vi "VIH Dialog - Enter Web or Mail address.vi"(11 "Type":enum16{"Website", "Email"}(ring)) -> (0 "OK out":bool, 2 "Subject out":string, 3 "Address out":string)   [LabVIEW 2014]
doc: "::: VI Helpeks :::\nCopyright (c) 2000-2026 Konstantin Shifershteyn. All rights reserved."
uses:
  <vilib>/Utility/miscctls.llb/LVSelectionTypeDef.ctl
panel:
  in  "Subject":string
  in  "%Cancel":bool
  in  "%OK":bool
  in  "Address":string caption="Website URL"
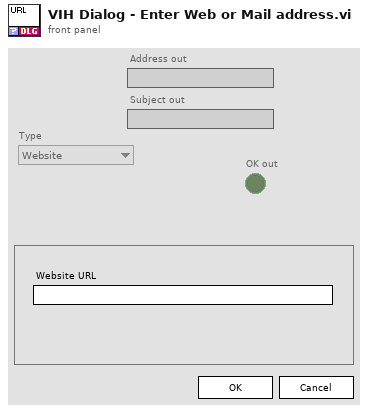
[diagram p1: front panel]
types:
  T1 = typedef "LVSelectionTypeDef.ctl" = cluster{"Selection Start":u32, "Selection End":u32}
  T2 = enum8{"Enabled", "Disabled", "Disabled and Grayed Out"}
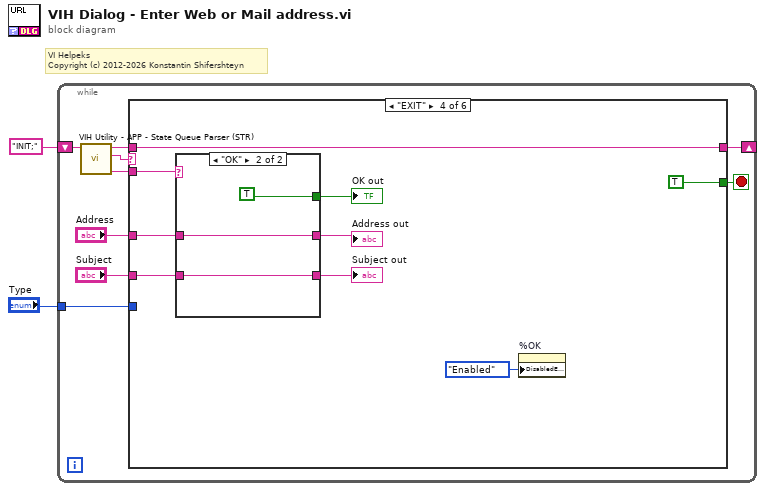
[diagram p0: block diagram]
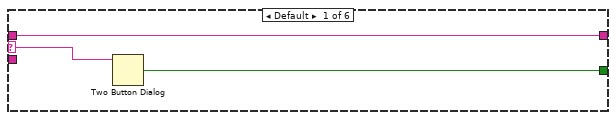
[diagram p2: hidden frame]
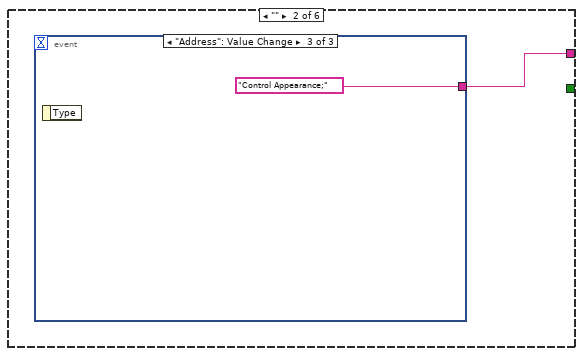
[diagram p3: hidden frame]
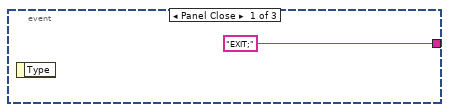
[diagram p4: hidden frame]
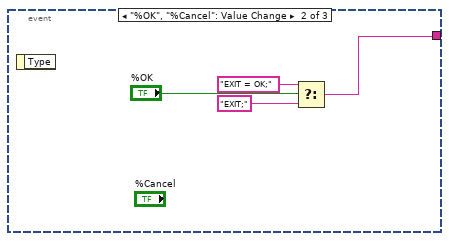
[diagram p5: hidden frame]
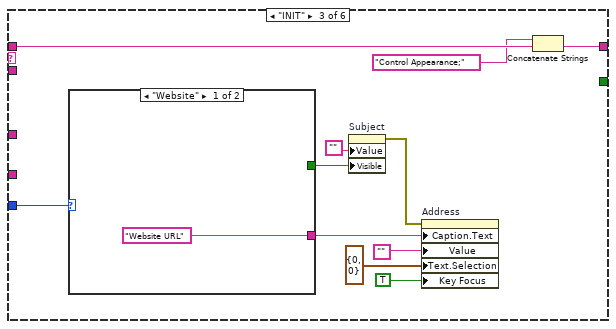
[diagram p6: hidden frame]
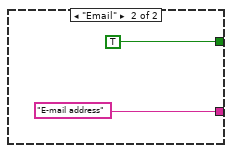
[diagram p7: hidden frame]
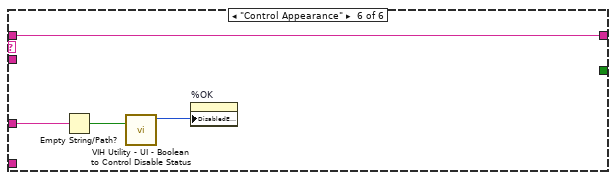
[diagram p10: hidden frame]
diagram:
  # "VI Helpeks\nCopyright (c) 2012-2026 Konstantin Shifershteyn"
  n1 = while {
    shift-right: [w9] -> _
    shift-left: "INIT;" -> [w11]
    tunnel: "Type" -> [w6]
    stop <- w7 stop-if-true
    n2 = call "VIH Utility - APP - State Queue Parser (STR).vi"("input queue"=w11) -> ("state parameters"=w4:string, "state"=w10:string, "remained queue"=w8:string)  [unwired: 5 in, 1 out]
    n3 = case shown="\"EXIT\"" w10 {
      selector: w10 -> [w13 _ _ _ _ _]
      tunnel: [w14 w15 w31 w44 w48 w52] -> w9
      tunnel: w8 -> [w14 _ w32 w44 w48 w52]
      tunnel: [w12 _ _ TRUE _ _] -> w7
      tunnel: w6 -> [_ _ w30 _ _ _]
      tunnel: "Address" -> [_ _ _ w40 _ w51]
      tunnel: w4 -> [_ _ _ w42 _ _]
      tunnel: "Subject" -> [_ _ _ w38 _ _]
      frame Default {
        n4 = Two Button Dialog(message=w13) -> (T button?=w12:bool)  [unwired: 2 in]
      }
      frame "" {
        n5 = event shown="[2] \"Address\": Value Change" {
          selector: _ -> [_ _ _]
          dyn-events: _ -> [_ _ _]
          timeout: _ -> [_ _ _]
          tunnel: ["EXIT;" w17 "Control Appearance;"] -> w15
          event Panel Close {
            n6 = event-data() -> ()  [unwired: 1 in, 1 out]
          }
          event "%OK", "%Cancel": Value Change {
            n7 = event-data() -> ()  [unwired: 1 in, 1 out]
            n8 = Select(t="EXIT = OK;", s="%OK", f="EXIT;") -> (s? t:f=w17:string)
          }
          event "Address": Value Change {
            n9 = event-data() -> ()  [unwired: 1 in, 1 out]
          }
        }
      }
      frame "INIT" {
        n10 = case shown="\"Website\"" w30 {
          tunnel: ["Website URL" "E-mail address"] -> w29
          tunnel: [_ TRUE] -> w25
          frame "Website" {
          }
          frame "Email" {
          }
        }
        n11 = property on="Subject" class="Str"("Value"="", "Visible"=w25) -> (error out=w23:errorcluster)  [unwired: 2 in, 1 out]
        n12 = property on="Address" class="Str"(error in=w23, "Caption.Text"=w29, "Value"="", "Text.Selection"=T1 {"Selection Start"=0, "Selection End"=0}, "Key Focus"=TRUE) -> ()  [unwired: 1 in, 2 out]
        n13 = Concatenate Strings("Control Appearance;" ("string"), w32) -> (w31:string)
      }
      frame "EXIT" {
        n14 = case shown="\"OK\"" w42 {
          tunnel: [_ w47] -> w41
          tunnel: w40 -> [_ w47]
          tunnel: [_ w46] -> w39
          tunnel: w38 -> [_ w46]
          tunnel: [_ TRUE] -> w37
          frame Default {
          }
          frame "OK" {
          }
        }
        "Address out" <- w41
        "Subject out" <- w39
        "OK out" <- w37
        n15 = property on="%OK" class="Bool"("DisabledEnum"=T2."Enabled" ("Disabled")) -> ()  [unwired: 2 in, 2 out]
      }
      frame "------------------------------ 1" {
      }
      frame "Control Appearance" {
        n16 = Empty String/Path?(string/path=w51) -> (empty?=w50:bool)
        n17 = call "VIH Utility - UI - Boolean to Control Disable Status.vi"("Status in"=w50) -> ("Control Disable if True"=w49:u8)  [unwired: 3 in, 1 out]
        n18 = property on="%OK" class="Bool"("DisabledEnum"=w49) -> ()  [unwired: 2 in, 2 out]
      }
    }
  }
